vi "Cleanup.vi"(8 "error in (no error)":errorcluster, 11 "Manager in":refnum<class "Manager.lvclass">) -> (0 "error out":errorcluster, 1 "Events":dbl, 2 "Wait Done":dbl)   [LabVIEW 2020, in "OOPanel.lvlib" / "Manager.lvclass"]
uses:
  Manager.lvclass
  Manager.lvclass/Manager.ctl
  Close Reason.ctl
  Panel/Panel.lvclass
  OOPanel.lvlib
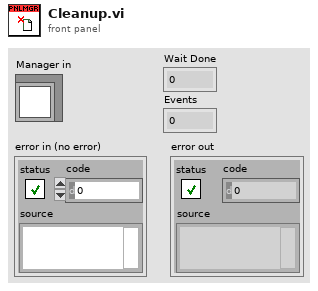
[diagram p1: front panel]
types:
  T1 = typedef "OOPanel.lvlib/Manager.lvclass/Ref Data.ctl" = cluster{"Created Panels":refnum<class "Panel.lvclass">[], "Subpanel Map":map{refnum<vi>, T2}}
  T2 = typedef "OOPanel.lvlib/Manager.lvclass/Subpanel Data.ctl" = cluster{"Panel":refnum<class "Panel.lvclass">, "Has Panel":bool, "Visible":bool}
  T3 = typedef "OOPanel.lvlib/Close Reason.ctl" = enum16{"Shutdown", "Close"}
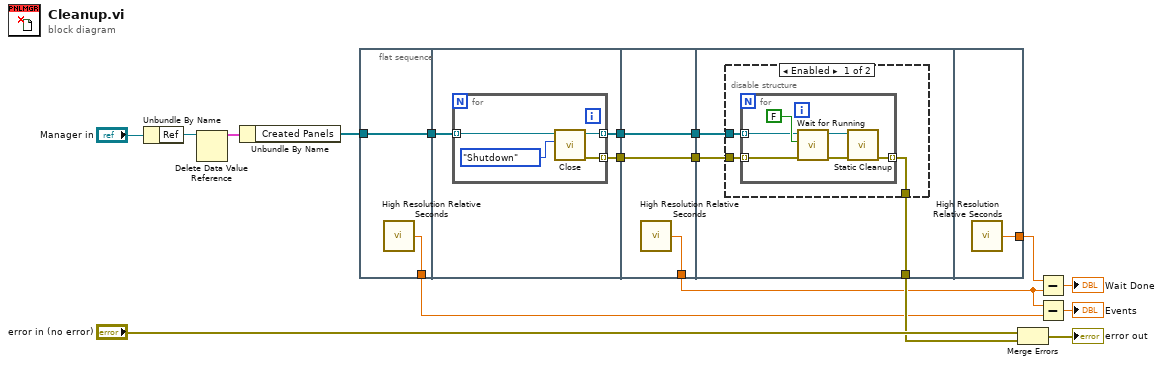
[diagram p0: block diagram]
diagram:
  n1 = Unbundle By Name("Manager in") -> ("Ref"=w15:refnum<data-value>)
  n2 = Delete Data Value Reference(data value reference=w15) -> (data value=w14:T1)  [unwired: 1 in, 1 out]
  n3 = Unbundle By Name(w14) -> ("Created Panels"=w12:refnum<class "Panel.lvclass">[])
  n4 = flat-sequence {
    tunnel: w12 -> [w19]
    tunnel: [w19] -> w8
    tunnel: [w18] -> w5
    tunnel: [w21] -> w9
    tunnel: w8 -> [w22]
    tunnel: [w20] -> w1
    tunnel: [w29] -> w10
    tunnel: w9 -> [w29]
    tunnel: [w28] -> w6
    tunnel: [w27] -> w2
    tunnel: w1 -> [w27]
    tunnel: [w32] -> w11
    tunnel: w10 -> [w31]
    tunnel: w2 -> [w30]
    tunnel: [w43] -> w7
    frame #0 {
      n5 = call <vilib>:"High Resolution Relative Seconds.vi"() -> ("relative seconds"=w18:dbl)
    }
    frame #1 {
      n6 = for {
        tunnel: w22 -> [w26] mode=indexing
        tunnel: [w24] -> w21 mode=indexing
        tunnel: [w23] -> w20 mode=indexing
        n7 = call "Close.vi"("Reason"=Close_Reason."Shutdown", "Panel in"=w26) -> ("error out"=w23:errorcluster, "Panel out"=w24:refnum<class "Panel.lvclass">)  [unwired: 8 in]
      }
    }
    frame #2 {
      n8 = call <vilib>:"High Resolution Relative Seconds.vi"() -> ("relative seconds"=w28:dbl)
    }
    frame #3 {
      n9 = disable-structure shown="Enabled" {
        disable-tunnel: [w35 w42] -> w32
        disable-tunnel: w31 -> [w34 _]
        disable-tunnel: w30 -> [w33 w42]
        frame Enabled {
          n10 = for {
            tunnel: [w37] -> w35 mode=indexing
            tunnel: w34 -> [w40] mode=indexing
            tunnel: w33 -> [w36] mode=indexing
            n11 = call "Wait for Running.vi"("error in (no error)"=w36, "Running"=FALSE, "Panel in"=w40) -> ("error out"=w38:errorcluster, "Panel out"=w39:refnum<class "Panel.lvclass">)  [unwired: 7 in]
            n12 = call "Static Cleanup.vi"("error in (no error)"=w38, "Panel in"=w39) -> ("error out"=w37:errorcluster)  [unwired: 9 in]
          }
        }
        frame Disabled {
        }
      }
    }
    frame #4 {
      n13 = call <vilib>:"High Resolution Relative Seconds.vi"() -> ("relative seconds"=w43:dbl)
    }
  }
  n14 = Merge Errors("error in (no error)", w11) -> (→"error out":errorcluster)
  n15 = Subtract(x=w7, y=w6) -> (x-y=→"Wait Done":dbl)
  n16 = Subtract(x=w6, y=w5) -> (x-y=→"Events":dbl)
